vi "Panel Resized.vi"(6 "Sizing Refnums":T2, 8 "error in (no error)":errorcluster, 9 "Origin":cluster{"H":i16, "V":i16}, 10 "NewBnds":T1, 11 "Size Constraints":cluster{"min tab width":i32, "w/h":dbl}) -> (0 "error out":errorcluster)   [LabVIEW 2017]
uses:
  <vilib>/Utility/miscctls.llb/LVRectTypeDef.ctl
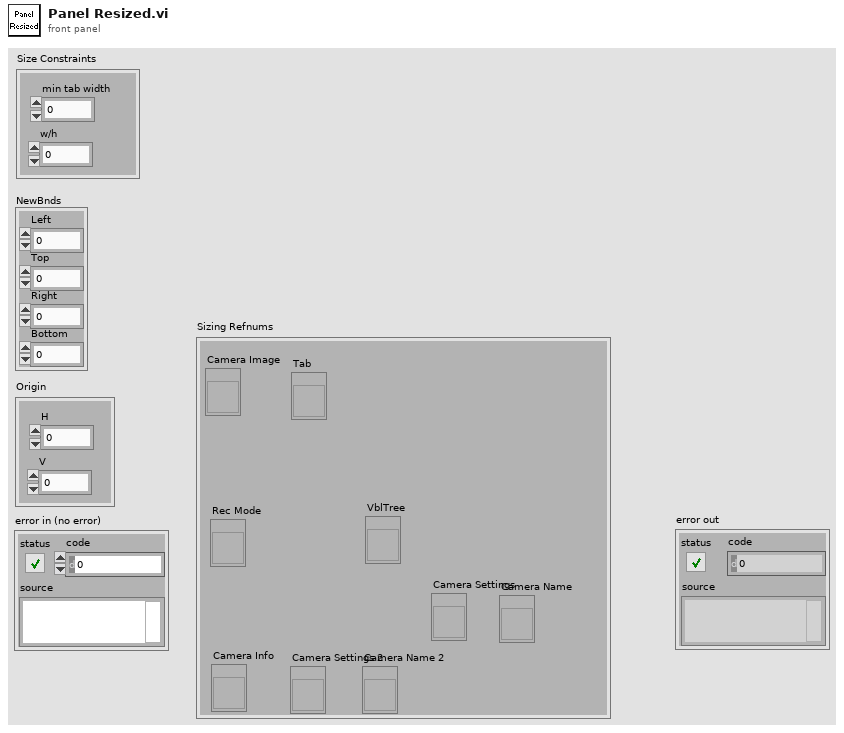
[diagram p1: front panel]
types:
  T1 = typedef "LVRectTypeDef.ctl" = cluster{"Left":i16, "Top":i16, "Right":i16, "Bottom":i16}
  T2 = cluster{"Camera Image":refnum<vi>, "Tab":refnum<vi>, "Rec Mode":refnum<vi>, "VblTree":refnum<vi>, "Camera Settings":refnum<vi>, "Camera Name":refnum<vi>, "Camera Info":refnum<vi>, "Camera Settings 2":refnum<vi>, "Camera Name 2":refnum<vi>}
  T3 = typedef "LVPositionTypeDef.ctl" = cluster{"Left":i32, "Top":i32}
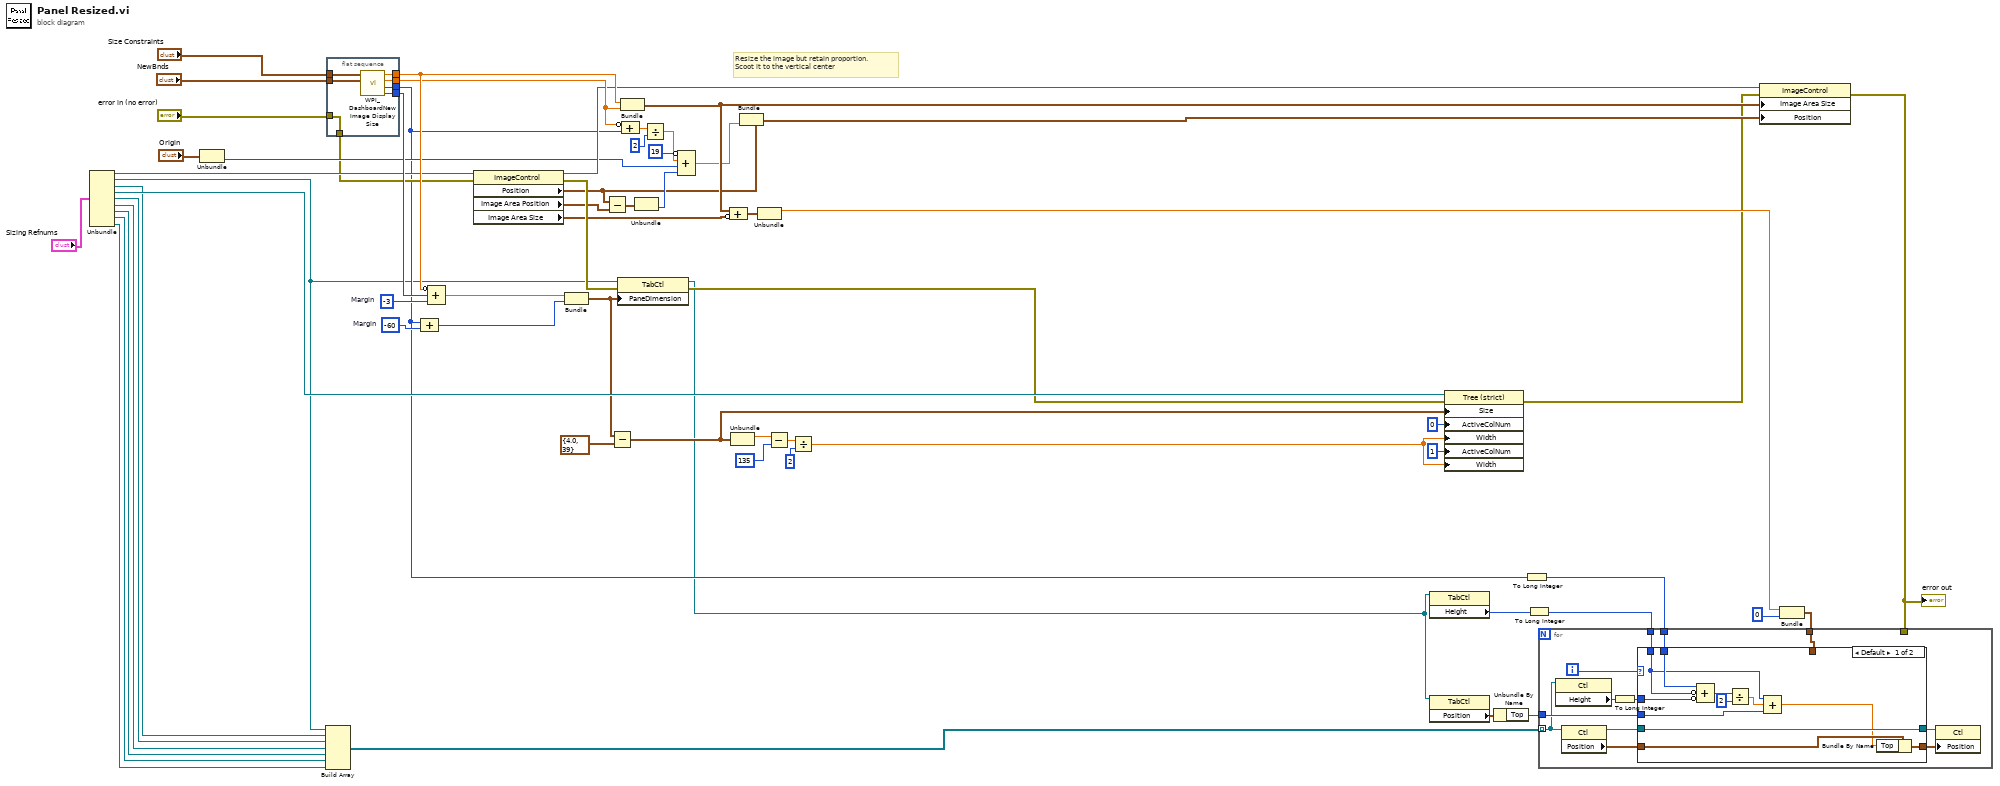
[diagram p0: block diagram]
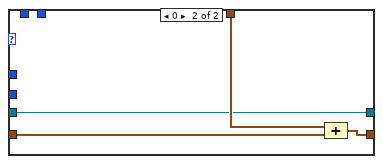
[diagram p2: hidden frame]
diagram:
  w8 = -60  # Margin
  w58 = -3  # Margin
  # "Resize the image but retain proportion.\nScoot it to the vertical center"
  n1 = Unbundle("Sizing Refnums") -> ("Camera Image"=w32:refnum<vi>, "Tab"=w5:refnum<vi>, "Rec Mode"=w16:refnum<vi>, "VblTree"=w27:refnum<vi>, "Camera Settings"=w15:refnum<vi>, "Camera Name"=w14:refnum<vi>, "Camera Info"=w13:refnum<vi>, "Camera Settings 2"=w12:refnum<vi>, "Camera Name 2"=w11:refnum<vi>)
  n2 = Unbundle("Origin") -> ("V"=w37:i16)  [unwired: 1 out]
  n3 = Build Array(w5, w16, w15, w14, w13, w12, w11) -> (w62:refnum<vi>[])
  n4 = flat-sequence {
    tunnel: "NewBnds" -> [w69]
    tunnel: "Size Constraints" -> [w68]
    tunnel: [w67] -> w54
    tunnel: [w66] -> w56
    tunnel: [w65] -> w7
    tunnel: [w64] -> w57
    tunnel: [w63] -> w30
    tunnel: "error in (no error)" -> [w63]
    frame #0 {
      n5 = call <vilib>:"WPI_DashboardNew Image Display Size.vi"("NewBnds"=w69, "Size Constraints"=w68) -> ("Window Width"=w67:i16, "Window Height"=w65:i16, "Height"=w66:dbl, "Width"=w64:dbl)  [unwired: 6 in]
    }
  }
  n6 = Compound Arithmetic op=unknown(w7, w8) -> (w6:i32)
  n7 = Compound Arithmetic op=ADD(invert w57, w54, w58) -> (w55:dbl)
  n8 = property class="ImageControl"(reference=w32, error in=w30) -> (reference out=w47:refnum<vi>, error out=w61:errorcluster, "Position"=w46:T3, "Image Area Position"=w41:cluster{"Left":i32, "Top":i32}, "Image Area Size"=w52:cluster{"Width":u32, "Height":u32})
  n9 = Bundle(w55, w6) -> (w23:cluster{dbl, i32})  [unwired: 1 in]
  n10 = Subtract(x=w46, y=w41) -> (x-y=w48:T3)
  n11 = Subtract(x=w23, y=cluster{dbl, i32} {4.0, 39}) -> (x-y=w18:cluster{dbl, i32})
  n12 = property class="TabCtl"(reference=w5, error in=w61, "PaneDimension"=w23) -> (reference out=w1:refnum<vi>, error out=w26:errorcluster)
  n13 = Bundle("Width"=w57, "Height"=w56) -> (w50:cluster{"Width":dbl, "Height":dbl})  [unwired: 1 in]
  n14 = Compound Arithmetic op=ADD(invert w56, w7) -> (w42:dbl)
  n15 = Unbundle(w48) -> ("Top"=w49:i32)  [unwired: 1 out]
  n16 = Divide(x=w42, y=2) -> (x/y=w44:dbl)
  n17 = Compound Arithmetic op=ADD(invert 19, w44, w37, w49) -> (w45:dbl)
  n18 = Compound Arithmetic op=ADD(w50, invert w52) -> (w53:cluster{"Width":dbl, "Height":dbl})
  n19 = Unbundle(w18) -> (w22:dbl)  [unwired: 1 out]
  n20 = Bundle(cluster=w46, "Top"=w45) -> (w51:T3)  [unwired: 1 in]
  n21 = Unbundle(w53) -> ("Width"=w59:dbl)  [unwired: 1 out]
  n22 = Subtract(x=w22, y=135 ("Active Cell:Active Column Number")) -> (x-y=w20:dbl)
  n23 = Divide(x=w20, y=2 ("Active Cell:Active Column Number")) -> (x/y=w17:dbl)
  n24 = property class="TabCtl"(reference=w1) -> ("Height"=w4:u32)  [unwired: 1 in, 2 out]
  n25 = property class="TabCtl"(reference=w1) -> ("Position"=w10:T3)  [unwired: 1 in, 2 out]
  n26 = property class="Tree (strict)"(reference=w27, error in=w26, "Size"=w18, "ActiveColNum"=0 ("Active Cell:Active Column Number"), "Width"=w17, "ActiveColNum"=1 ("Active Cell:Active Column Number"), "Width"=w17) -> (error out=w25:errorcluster)  [unwired: 1 out]
  n27 = Unbundle By Name(w10) -> ("Top"=w9:i32)
  n28 = To Long Integer(number=w7) -> (32bit integer=w2:i32)
  n29 = To Long Integer(number=w4) -> (32bit integer=w3:i32)
  n30 = property class="ImageControl"(reference=w47, error in=w25, "Image Area Size"=w50, "Position"=w51) -> (error out=w36:errorcluster)  [unwired: 1 out]
  "error out" <- w36
  n31 = Bundle("Width"=w59, 0) -> (w40:cluster{"Width":dbl, i32})  [unwired: 1 in]
  n32 = for {
    tunnel: w62 -> [w74] mode=indexing
    tunnel: w40 -> [w80]
    tunnel: w36 -> [_]
    tunnel: w9 -> [w75]
    tunnel: w2 -> [w72]
    tunnel: w3 -> [w71]
    i -> [w81]
    n33 = property class="Ctl"(reference=w74) -> ("Height"=w73:u32)  [unwired: 1 in, 2 out]
    n34 = property class="Ctl"(reference=w74) -> (reference out=w77:refnum<vi>, "Position"=w79:T3)  [unwired: 1 in, 1 out]
    n35 = To Long Integer(number=w73) -> (32bit integer=w70:i32)
    n36 = case shown="Default" w81 {
      tunnel: w80 -> [_ w96]
      tunnel: w79 -> [w91 w95]
      tunnel: [w92 w94] -> w78
      tunnel: w77 -> [w90 w93]
      tunnel: [w90 w93] -> w76
      tunnel: w75 -> [w82 _]
      tunnel: w70 -> [w87 _]
      tunnel: w72 -> [w88 _]
      tunnel: w71 -> [w83 _]
      frame Default {
        n37 = Compound Arithmetic op=ADD(w88, invert w83, invert w87) -> (w86:i32)
        n38 = Divide(x=w86, y=u32 2) -> (x/y=w84:dbl)
        n39 = Compound Arithmetic op=ADD(w83, w84, w82) -> (w89:dbl)
        n40 = Bundle By Name(cluster=w91, "Top"=w89) -> (w92:T3)
      }
      frame 0 {
        n41 = Compound Arithmetic op=ADD(w96, w95) -> (w94:cluster{dbl, i32})
      }
    }
    n42 = property class="Ctl"(reference=w76, "Position"=w78) -> ()  [unwired: 1 in, 2 out]
  }
